vi "VIH UI - Get Icon 32x32 for Tree Item.vi"(6 "cmd (get)":enum16{"get", "reset"}(ring), 8 "error in":errorcluster, 9 "# Items (1)":i32=1, 10 "Item Name":string, 11 "Tree Item Tag":string) -> (0 "error out":errorcluster, 2 "Item Icon":picture)   [LabVIEW 2014]
doc: "::: VI Helpeks :::\nCopyright (c) 2000-2026 Konstantin Shifershteyn. All rights reserved."
uses:
  VIH Project Tree Typedef - Tree Item Type.ctl
panel:
  in  "DefIcon - Default Palette":picture
  in  "DefIcon - MultiItems":picture
  in  "DefIcon - Project Files":picture
  in  "DefIcon - Project":picture
  in  "DefIcon - Group":picture
  in  "DefIcon - Default Built-In":picture
  in  "DefIcon - Default VI":picture
  in  "DefIcon - Text":picture
  in  "DefIcon - Image":picture
  in  "DefIcon - Any File":picture
  in  "DefIcon - Invalid":picture
  in  "DefIcon - HTML":picture
  in  "DefIcon - VI Helpeks":picture
  # "VI Helpeks\nCopyright (c) 2012-2026 Konstantin Shifershteyn"
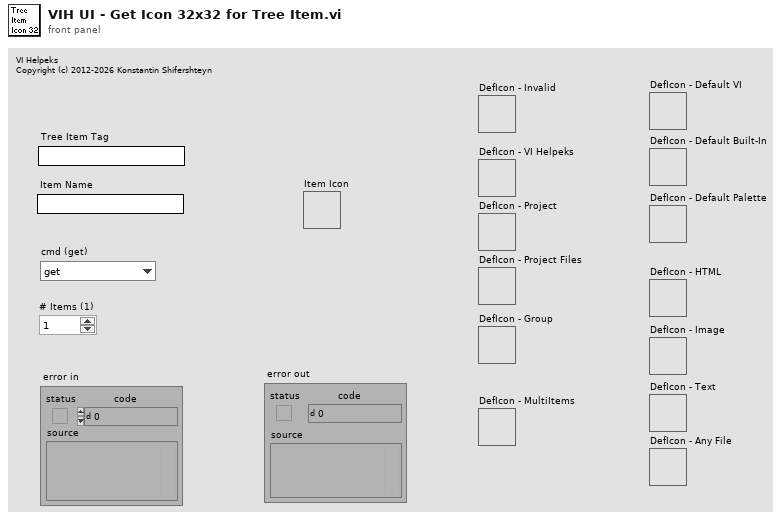
[diagram p1: front panel]
types:
  T1 = enum32{"<Invalid>", "Project", "Proj Files", "Proj Rules", "File Group", "Rule Group", "Any File", "LV Func", ".mnu", ".mnu (dyn)", ".vi", ".vi (dyn)", ".vit", ".vit (dyn)", ".ctl", ".ctl (dyn)", ".ctt", ".ctt (dyn)", "polyVI", "polyVI (dyn)", "expVI", "expVI (dyn)", "HTML", "PolyVI Inst"}
  T2 = typedef "VIH Project Tree Typedef - Tree Item Type.ctl" = enum32{"<Invalid>", "Project", "Proj Files", "Proj Rules", "File Group", "Rule Group", "Any File", "LV Func", ".mnu", ".mnu (dyn)", ".vi", ".vi (dyn)", ".vit", ".vit (dyn)", ".ctl", ".ctl (dyn)", ".ctt", ".ctt (dyn)", "polyVI", "polyVI (dyn)", "expVI", "expVI (dyn)", "HTML", "PolyVI Inst"}
  T3 = cluster{"Item Type":T2, "Item File Path":path, "Item Name":string}[]
  T4 = typedef "imagedata.ctl" = cluster{"image type":i32, "image depth":i32, "image":u8[], "mask":u8[], "colors":u32[], "Rectangle":cluster{"left":i16, "top":i16, "right":i16, "bottom":i16}}
  T5 = cluster{"Item Type":T2, "Item File Path":path, "Item Name":string}
  T6 = typedef "Palette Menu.lvlib/Palette Data.ctl" = cluster{"display name":string, "view format":T7, "palette width":i16, "items":T8, "256 color icon":picture, "B&W color icon":picture, "help information":T10, "palette description":string, "synchronize information":T11}
  T7 = typedef "Palette Menu.lvlib/View Format.ctl" = u16
  T8 = typedef "Palette Menu.lvlib/Items.ctl" = T9[]
  T9 = typedef "Palette Menu.lvlib/Item.ctl" = cluster{"item path":path, "library path (.lvlib)":path, "use default lvlib palette":bool, "short name":string, "place VI contents":bool, "hide synchronized item":bool, "reserve spot for synch item":bool, "configure when placing VI contents":bool}
  T10 = typedef "Palette Menu.lvlib/Help Info.ctl" = cluster{"help tag":string, "help file path ":path}
  T11 = typedef "Palette Menu.lvlib/Synchronize Info.ctl" = cluster{"synchronize with directory":bool, "synchronize directory path":path}
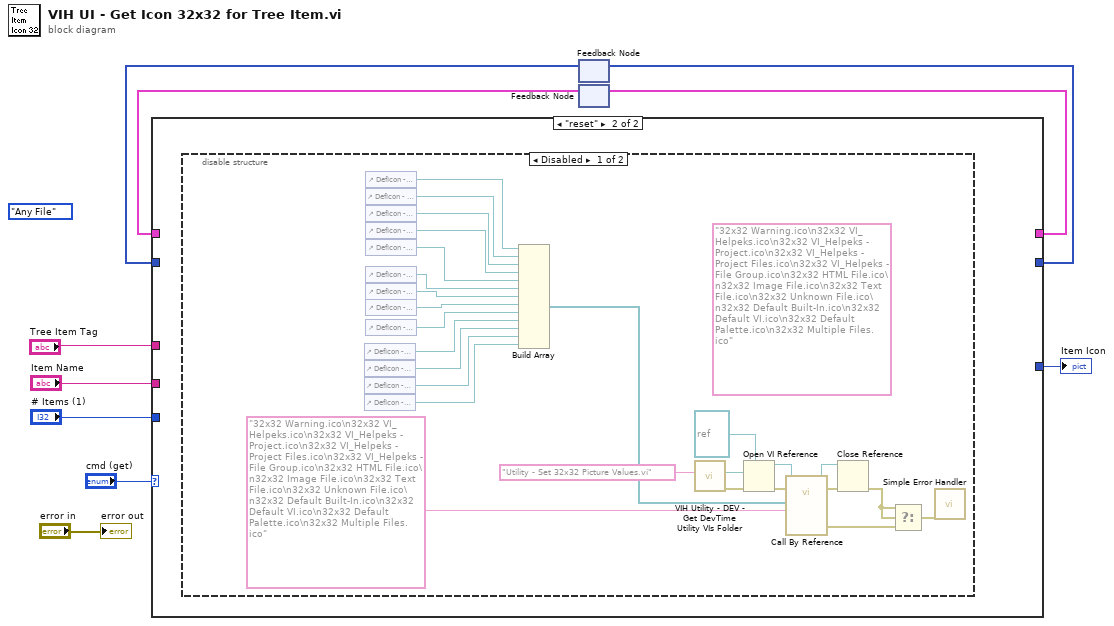
[diagram p0: block diagram]
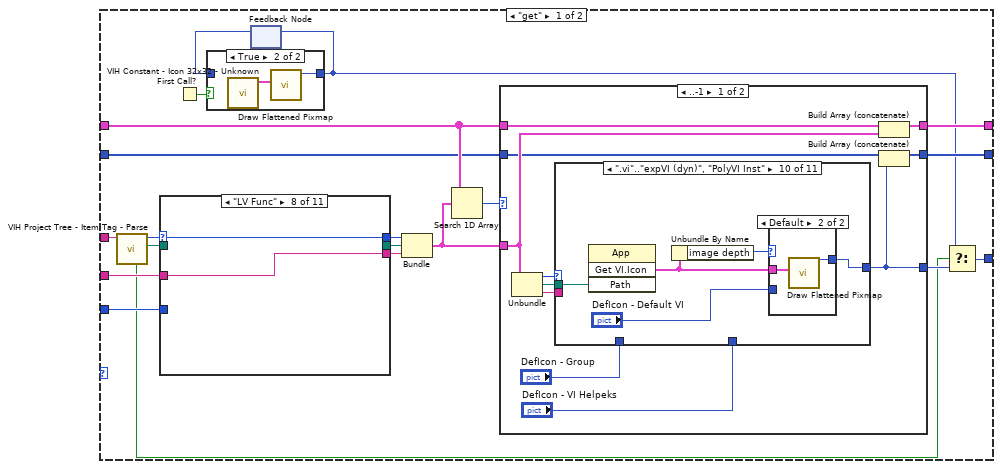
[diagram p2: hidden frame]
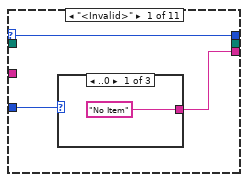
[diagram p4: hidden frame]
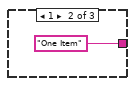
[diagram p5: hidden frame]
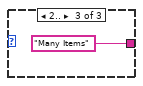
[diagram p6: hidden frame]
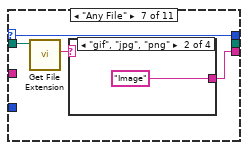
[diagram p12: hidden frame]
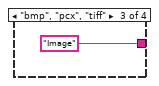
[diagram p14: hidden frame]
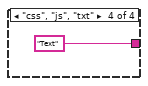
[diagram p15: hidden frame]
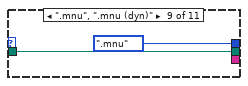
[diagram p16: hidden frame]
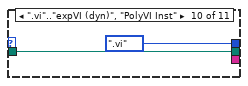
[diagram p17: hidden frame]
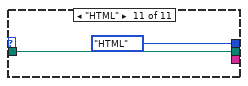
[diagram p18: hidden frame]
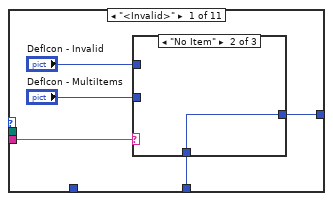
[diagram p19: hidden frame]
diagram:
  (unwired) T1."Any File" ("Item Type")
  n1 = feedback #1() -> (w6:picture[])  [unwired: 1 in]
  n2 = feedback #2() -> (w7:T3)  [unwired: 1 in]
  n3 = case shown="\"reset\"" "cmd (get)" {
    tunnel: "Tree Item Tag" -> [w30 _]
    tunnel: "Item Name" -> [w22 _]
    tunnel: [w27 _] -> w8
    tunnel: w7 -> [w26 _]
    tunnel: w6 -> [w25 _]
    tunnel: [w24 _] -> w5
    tunnel: [w13 _] -> w3
    tunnel: "# Items (1)" -> [w17 _]
    frame "get" {
      n4 = call "VIH Project Tree - Item Tag - Parse.vi"("Tree Item Tag"=w30) -> ("Item File Path"=w21:path, "Item Type"=w23:T2, "Not Found"=w11:bool)  [unwired: 8 in]
      n5 = case shown="\"LV Func\"" w23 {
        selector: w23 -> [w36 w40 w41 w42 w43 w44 w48 w53 _ _ _]
        tunnel: [w36 w40 w41 w42 w43 w44 w48 w53 VIH_Project_Tree_Typedef_-_Tree_Item_Type.".mnu" ("Item Type") VIH_Project_Tree_Typedef_-_Tree_Item_Type.".vi" ("Item Type") VIH_Project_Tree_Typedef_-_Tree_Item_Type."HTML" ("Item Type")] -> w20
        tunnel: [w34 _ _ _ _ _ w45 w52 _ _ _] -> w18
        tunnel: w22 -> [_ _ _ _ _ _ _ w52 _ _ _]
        tunnel: [_ _ _ _ _ _ _ _ w54 w56 w58] -> w19
        tunnel: w21 -> [_ _ _ _ _ _ w47 _ w54 w56 w58]
        tunnel: w17 -> [w35 _ _ _ _ _ _ _ _ _ _]
        frame "<Invalid>" {
          n6 = case shown="..0" w35 {
            tunnel: ["No Item" "One Item" "Many Items"] -> w34
            frame ..0 {
            }
            frame 1 {
            }
            frame 2.. {
            }
          }
        }
        frame "Project" {
        }
        frame "Proj Files" {
        }
        frame "Proj Rules" {
        }
        frame "File Group" {
        }
        frame "Rule Group" {
        }
        frame "Any File" {
          n7 = call <vilib>:"Get File Extension.vi"("file"=w47) -> ("lowercase file extension"=w46:string)  [unwired: 7 in, 3 out]
          n8 = case shown="\"gif\", \"jpg\", \"png\"" w46 {
            tunnel: [_ "Image" "Image" "Text"] -> w45
            frame Default {
            }
            frame "gif", "jpg", "png" {
            }
            frame "bmp", "pcx", "tiff" {
            }
            frame "css", "js", "txt" {
            }
          }
        }
        frame "LV Func" {
        }
        frame ".mnu", ".mnu (dyn)" {
        }
        frame ".vi".."expVI (dyn)", "PolyVI Inst" {
        }
        frame "HTML" {
        }
      }
      n9 = First Call?() -> (First Call?: T/F=w15:bool)
      n10 = feedback #3() -> (w16:picture)  [unwired: 1 in]
      n11 = case shown="True" w15 {
        tunnel: [w31 w32] -> w12
        tunnel: w16 -> [w31 _]
        frame False {
        }
        frame True {
          n12 = call "VIH Constant - Icon 32x32 - Unknown.vi"() -> ("image data"=w33:T4)  [unwired: 11 in]
          n13 = call <vilib>:"Draw Flattened Pixmap.vi"("image data"=w33) -> ("new picture"=w32:picture)  [unwired: 8 in]
        }
      }
      n14 = feedback-in #3(w12) -> ()
      n15 = Bundle("Item Type"=w20, "Item File Path"=w19, "Item Name"=w18) -> (w28:T5)  [unwired: 1 in]
      n16 = Search 1D Array(1D array=w26, element=w28) -> (index of element=w29:i32)  [unwired: 1 in]
      n17 = case shown="..-1" w29 {
        selector: w29 -> [_ w119]
        tunnel: w28 -> [w68 _]
        tunnel: w26 -> [w70 w120]
        tunnel: [w69 w120] -> w27
        tunnel: w25 -> [w67 w118]
        tunnel: [w66 w118] -> w24
        tunnel: [w62 w117] -> w14
        frame ..-1 {
          n18 = Unbundle(w68) -> ("Item Type"=w65:T2, "Item File Path"=w64:path, "Item Name"=w63:string)
          n19 = case shown="\".vi\"..\"expVI (dyn)\", \"PolyVI Inst\"" w65 {
            tunnel: w63 -> [w75 _ _ _ _ _ w88 w93 _ _ _]
            tunnel: w64 -> [_ _ _ _ _ _ _ _ w106 w112 _]
            tunnel: [w74 "DefIcon - Project" "DefIcon - Project Files" w81 w82 w83 w87 w95 w107 w109 "DefIcon - HTML"] -> w62
            tunnel: "DefIcon - VI Helpeks" -> [w72 _ _ w81 _ w83 _ _ _ _ _]
            tunnel: "DefIcon - Group" -> [_ _ _ _ w82 _ _ _ _ _ _]
            frame "<Invalid>" {
              n20 = case shown="\"No Item\"" w75 {
                tunnel: [w76 w77 w78] -> w74
                tunnel: "DefIcon - Invalid" -> [w76 _ _]
                tunnel: w72 -> [_ w77 _]
                tunnel: "DefIcon - MultiItems" -> [_ _ w78]
                frame "One Item", Default {
                }
                frame "No Item" {
                }
                frame "Many Items" {
                }
              }
            }
            frame "Project" {
            }
            frame "Proj Files" {
            }
            frame "Proj Rules" {
            }
            frame "File Group" {
            }
            frame "Rule Group" {
            }
            frame "Any File" {
              n21 = case shown="\"Image\", \"Picture\"" w88 {
                tunnel: [w89 w90 w91] -> w87
                tunnel: "DefIcon - Any File" -> [w89 _ _]
                tunnel: "DefIcon - Image" -> [_ w90 _]
                tunnel: "DefIcon - Text" -> [_ _ w91]
                frame Default {
                }
                frame "Image", "Picture" {
                }
                frame "Text" {
                }
              }
            }
            frame "LV Func" {
              n22 = call "VIH Platform - LabVIEW - Palette - Get Item Image.vi"("Palette Item Name"=w93) -> ("Palette Item Icon"=w92:T4)  [unwired: 8 in, 2 out]
              n23 = Unbundle By Name(w92) -> ("image depth"=w96:i32)
              n24 = case shown="Default" w96 {
                tunnel: w92 -> [_ w99]
                tunnel: [w97 w98] -> w95
                tunnel: "DefIcon - Default Built-In" -> [w97 _]
                frame 0 {
                }
                frame Default {
                  n25 = call <vilib>:"Draw Flattened Pixmap.vi"("image data"=w99) -> ("new picture"=w98:picture)  [unwired: 8 in]
                }
              }
            }
            frame ".mnu", ".mnu (dyn)" {
              n26 = call "VIH HelpGen - Palette - Read Palette (non-palette allowed).vi"("Palette Path"=w106) -> ("palette data"=w105:T6)  [unwired: 8 in, 2 out]
              n27 = Unbundle By Name(w105) -> ("256 color icon"=w102:picture)
              n28 = call "Empty Picture"() -> ("empty picture"=w101:picture)
              n29 = Equal?(x=w101, y=w102) -> (x = y?=w100:bool)
              n30 = Select(t="DefIcon - Default Palette", s=w100, f=w102) -> (s? t:f=w103:picture)
              n31 = call "VIH HelpGen - Image - Add Transparency to Icon Picture.vi"("2D Picture"=w103) -> ("2D Picture out"=w107:picture)  [unwired: 10 in]
            }
            frame ".vi".."expVI (dyn)", "PolyVI Inst" {
              n32 = invoke class="App" method="Get VI.Icon"("Path"=w112) -> ("Get VI.Icon"=w110:T4)  [unwired: 3 in, 3 out]
              n33 = Unbundle By Name(w110) -> ("image depth"=w111:i32)
              n34 = case shown="Default" w111 {
                tunnel: w110 -> [_ w115]
                tunnel: [w113 w114] -> w109
                tunnel: "DefIcon - Default VI" -> [w113 _]
                frame 0 {
                }
                frame Default {
                  n35 = call <vilib>:"Draw Flattened Pixmap.vi"("image data"=w115) -> ("new picture"=w114:picture)  [unwired: 8 in]
                }
              }
            }
            frame "HTML" {
            }
          }
          n36 = Build Array (concatenate)(w70, w68) -> (w69:T3)
          n37 = Build Array (concatenate)(w67, w62) -> (w66:picture[])
        }
        frame 0.. {
          n38 = Index Array(array=w118, index=w119) -> (element=w117:picture)
        }
      }
      n39 = Select(t=w12, s=w11, f=w14) -> (s? t:f=w13:picture)
    }
    frame "reset" {
      n40 = disable-structure shown="Disabled" {
        frame Disabled {
          (unwired) "32x32 Warning.ico\n32x32 VI_Helpeks.ico\n32x32 VI_Helpeks - Project.ico\n32x32 VI_Helpeks - Project Files.ico\n32x32 VI_Helpeks - File Group.ico\n32x32 HTML File.ico\n32x32 Image File.ico\n32x32 Text File.ico\n32x32 Unknown File.ico\n32x32 Default Built-In.ico\n32x32 Default VI.ico\n32x32 Default Palette.ico\n32x32 Multiple Files.ico" ("Icon Names")
          n41 = control-ref of="DefIcon - Default Built-In"() -> (w140:refnum<vi>)
          n42 = control-ref of="DefIcon - Default VI"() -> (w139:refnum<vi>)
          n43 = control-ref of="DefIcon - Default Palette"() -> (w121:refnum<vi>)
          n44 = control-ref of="DefIcon - MultiItems"() -> (w123:refnum<vi>)
          n45 = control-ref of="DefIcon - Invalid"() -> (w144:refnum<vi>)
          n46 = control-ref of="DefIcon - VI Helpeks"() -> (w146:refnum<vi>)
          n47 = control-ref of="DefIcon - Project"() -> (w137:refnum<vi>)
          n48 = control-ref of="DefIcon - Project Files"() -> (w136:refnum<vi>)
          n49 = control-ref of="DefIcon - Group"() -> (w138:refnum<vi>)
          n50 = control-ref of="DefIcon - HTML"() -> (w145:refnum<vi>)
          n51 = control-ref of="DefIcon - Image"() -> (w143:refnum<vi>)
          n52 = control-ref of="DefIcon - Text"() -> (w141:refnum<vi>)
          n53 = control-ref of="DefIcon - Any File"() -> (w142:refnum<vi>)
          n54 = Build Array(w144, w146, w137, w136, w138, w145, w143, w141, w142, w140, w139, w121, w123) -> (w125:refnum<vi>[])
          n55 = call "VIH Utility - DEV - Get DevTime Utility VIs Folder.vi"("Utility VI Name"="Utility - Set 32x32 Picture Values.vi") -> ("error out"=w130:errorcluster, "Utility VIs Path"=w131:path)  [unwired: 8 in, 1 out]
          n56 = Open VI Reference(type specifier VI Refnum (for type only)=refnum<vi> refnum, vi path=w131, error in (no error)=w130) -> (vi reference=w128:refnum<vi>, error out=w127:errorcluster)  [unwired: 3 in]
          n57 = call-by-ref "?"(reference=w128, error in=w127, "Icon Names"="32x32 Warning.ico\n32x32 VI_Helpeks.ico\n32x32 VI_Helpeks - Project.ico\n32x32 VI_Helpeks - Project Files.ico\n32x32 VI_Helpeks - File Group.ico\n32x32 HTML File.ico\n32x32 Image File.ico\n32x32 Text File.ico\n32x32 Unknown File.ico\n32x32 Default Built-In.ico\n32x32 Default VI.ico\n32x32 Default Palette.ico\n32x32 Multiple Files.ico", "Picture Refnums"=w125) -> (reference out=w133:refnum<vi>, error out=w132:errorcluster, 0:"error out"=w135:errorcluster)  [unwired: 9 in]
          n58 = Close Reference(reference=w133, error in (no error)=w132) -> (error out=w122:errorcluster)
          n59 = Select(t=w122, s=w122, f=w135) -> (s? t:f=w134:errorcluster)
          n60 = call <vilib>:"Simple Error Handler.vi"("error in (no error)"=w134) -> ()  [unwired: 4 in, 5 out]
        }
        frame Enabled {
        }
      }
    }
  }
  "Item Icon" <- w3
  n61 = feedback-in #1(w5) -> ()
  n62 = feedback-in #2(w8) -> ()
  "error out" <- "error in"
